vi "Parse Call Process Param.vi"(8 "error in (no error)":errorcluster caption="에러 입력(에러 없음)", 10 "JSON string":string, 11 "Instrument Manager 입력":refnum<class "Instrument Manager.lvclass">) -> (0 "error out":errorcluster caption="에러 출력", 1 "NR Call Process Param":T2, 2 "NR Call Process Param":T1, 3 "Instrument Manager 출력":refnum<class "Instrument Manager.lvclass">)   [LabVIEW 2023, in "Instrument Manager.lvclass"]
uses:
  Instrument Manager.lvclass
  Type Definition/NR Call Process Param.ctl
  Module/ANRITSU Call Box/Type Definition/NR Modulation Type.ctl
  Param Definition/Call Process Param.ctl
  Instrument Manager.lvclass/Instrument Manager.ctl
  Module/ANRITSU Call Box/ANRITSU Call Box.lvlib
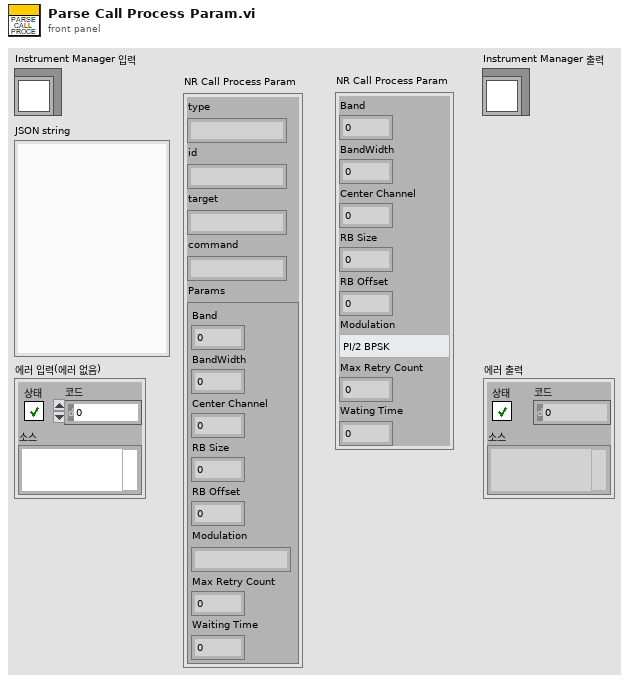
[diagram p1: front panel]
types:
  T1 = typedef "Instrument Manager.lvclass/Call Process Param.ctl" = cluster{"type":string, "id":string, "target":string, "command":string, "Params":cluster{"Band":u32, "BandWidth":u32, "Center Channel":u32, "RB Size":i32, "RB Offset":i32, "Modulation":string, "Max Retry Count":i32, "Waiting Time":i32}}
  T2 = typedef "NR Call Process Param.ctl" = cluster{"Band":u32, "BandWidth":u32, "Center Channel":u32, "RB Size":i32, "RB Offset":i32, "Modulation":T3, "Max Retry Count":i32, "Wating Time":i32}
  T3 = typedef "ANRITSU Call Box.lvlib/NR Modulation Type.ctl" = enum16{"PI/2 BPSK", "QPSK", "16QAM", "64QAM", "256QAM"}
  T4 = cluster{"Band":u32, "BandWidth":u32, "Center Channel":u32, "RB Size":i32, "RB Offset":i32, "Modulation":string, "Max Retry Count":i32, "Waiting Time":i32}
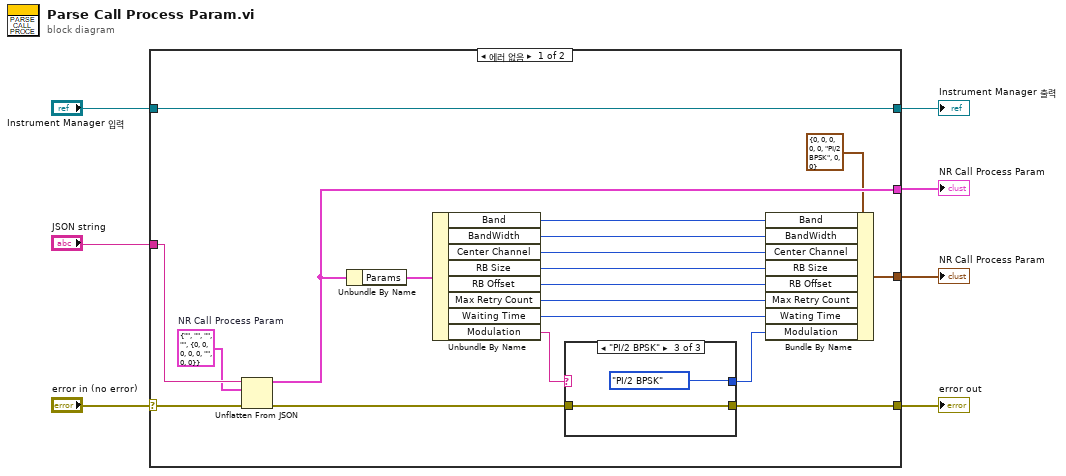
[diagram p0: block diagram]
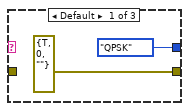
[diagram p2: hidden frame]
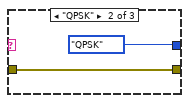
[diagram p3: hidden frame]
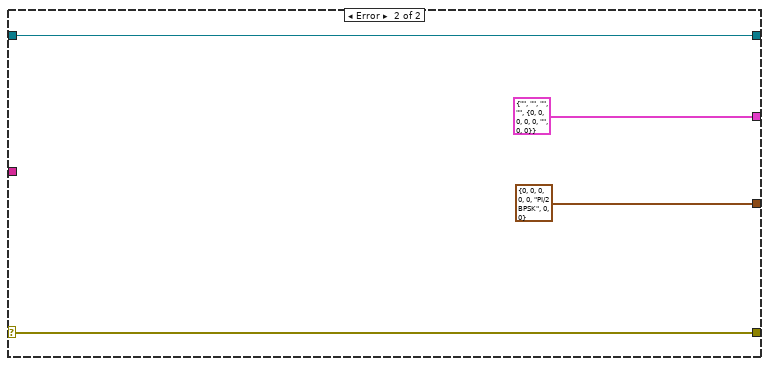
[diagram p4: hidden frame]
diagram:
  n1 = case shown="에러 없음" "error in (no error)" {
    selector: "error in (no error)" -> [w25 w36]
    tunnel: [w12 w36] -> w6
    tunnel: [w26 w35] -> w4
    tunnel: "Instrument Manager 입력" -> [w26 w35]
    tunnel: "JSON string" -> [w24 _]
    tunnel: [w21 T1 {"type"="", "id"="", "target"="", "command"="", "Params"={"Band"=0, "BandWidth"=0, "Center Channel"=0, "RB Size"=0, "RB Offset"=0, "Modulation"="", "Max Retry Count"=0, "Waiting Time"=0}} ("NR Call Process Param")] -> w2
    tunnel: [w13 T2 {"Band"=0, "BandWidth"=0, "Center Channel"=0, "RB Size"=0, "RB Offset"=0, "Modulation"=enum."PI/2 BPSK", "Max Retry Count"=0, "Wating Time"=0} ("NR Call Process Param")] -> w1
    frame No Error {
      w23 = T1 {"type"="", "id"="", "target"="", "command"="", "Params"={"Band"=0, "BandWidth"=0, "Center Channel"=0, "RB Size"=0, "RB Offset"=0, "Modulation"="", "Max Retry Count"=0, "Waiting Time"=0}}  # NR Call Process Param
      n2 = Unflatten From JSON(JSON string=w24, type and defaults=w23, error in (no error)=w25) -> (value=w21:T1, error out=w14:errorcluster)  [unwired: 4 in]
      n3 = Unbundle By Name(w21) -> ("Params"=w22:T4)
      n4 = Unbundle By Name(w22) -> ("Band"=w19:u32, "BandWidth"=w18:u32, "Center Channel"=w17:u32, "RB Size"=w15:i32, "RB Offset"=w16:i32, "Max Retry Count"=w8:i32, "Waiting Time"=w9:i32, "Modulation"=w11:string)
      n5 = case shown="\"PI/2 BPSK\"" w11 {
        tunnel: w14 -> [_ w30 w32]
        tunnel: [errorcluster {"status"=TRUE, "code"=0, "source"=""} ("error out") w30 w32] -> w12
        tunnel: [NR_Modulation_Type."QPSK" ("Modulation") NR_Modulation_Type."QPSK" ("Modulation") NR_Modulation_Type."PI/2 BPSK" ("Modulation")] -> w10
        frame Default {
        }
        frame "QPSK" {
        }
        frame "PI/2 BPSK" {
        }
      }
      n6 = Bundle By Name(cluster=T2 {"Band"=0, "BandWidth"=0, "Center Channel"=0, "RB Size"=0, "RB Offset"=0, "Modulation"=enum."PI/2 BPSK", "Max Retry Count"=0, "Wating Time"=0} ("NR Call Process Param"), "Band"=w19, "BandWidth"=w18, "Center Channel"=w17, "RB Size"=w15, "RB Offset"=w16, "Max Retry Count"=w8, "Wating Time"=w9, "Modulation"=w10) -> (w13:T2)
    }
    frame Error {
    }
  }
  "error out" <- w6
  "Instrument Manager 출력" <- w4
  "NR Call Process Param" <- w2
  "NR Call Process Param" <- w1
